vi "Set Cell Data.vi"(4 "Ref. Value":string, 6 "Ref. Header":string, 8 "error in (no error)":errorcluster, 9 "Cell Data":string, 10 "Cell Header":string, 11 "SLL Table in":refnum<class "SLL Table.lvclass">) -> (0 "error out":errorcluster, 3 "SLL Table out":refnum<class "SLL Table.lvclass">)   [LabVIEW 2016, in "SLL Table.lvclass"]
doc: "Set a specific cell value with respect to reference header and value."
uses:
  SLL Table.lvclass
  SLL Table.lvclass/SLL Table.ctl
panel:
  out "Header Present?":bool
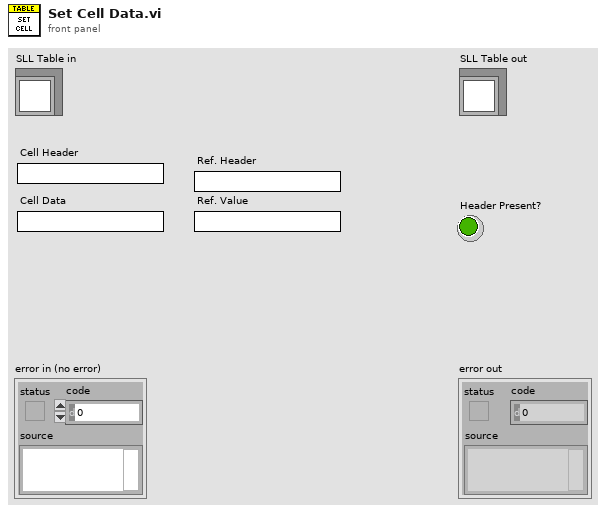
[diagram p1: front panel]
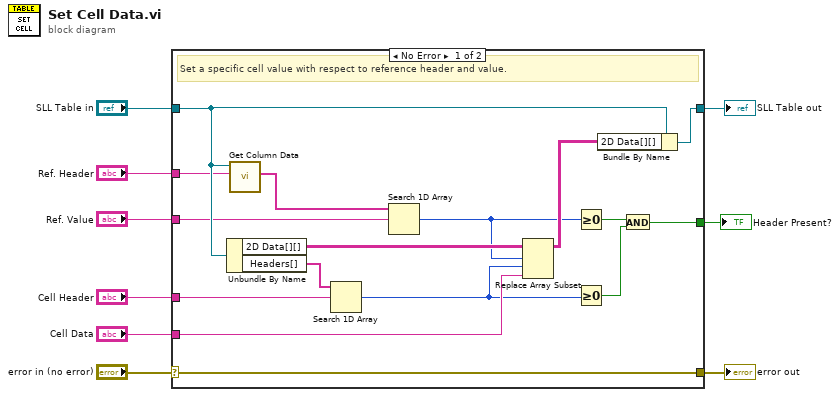
[diagram p0: block diagram]
diagram:
  n1 = case shown="No Error" "error in (no error)" {
    selector: "error in (no error)" -> [w25 w27]
    tunnel: [w25 w27] -> w8
    tunnel: [w18 w26] -> w6
    tunnel: "SLL Table in" -> [w19 w26]
    tunnel: "Cell Header" -> [w22 _]
    tunnel: "Cell Data" -> [w20 _]
    tunnel: "Ref. Header" -> [w16 _]
    tunnel: "Ref. Value" -> [w15 _]
    tunnel: [w10 _] -> w1
    frame No Error {
      # "Set a specific cell value with respect to reference header and value."
      n2 = Unbundle By Name(w19) -> ("2D Data[][]"=w21:string[][], "Headers[]"=w23:string[])
      n3 = call "Get Column Data.vi"("Header"=w16, "SLL Table in"=w19) -> ("Data[]"=w24:string[])  [unwired: 6 in, 3 out]
      n4 = Search 1D Array(1D array=w23, element=w22) -> (index of element=w13:i32)  [unwired: 1 in]
      n5 = Search 1D Array(1D array=w24, element=w15) -> (index of element=w14:i32)  [unwired: 1 in]
      n6 = Replace Array Subset(array=w21, new element=w20, index (row)=w14, index (col)=w13) -> (w17:string[][])
      n7 = Greater Or Equal To 0?(x=w14) -> (x >= 0?=w12:bool)
      n8 = Greater Or Equal To 0?(x=w13) -> (x >= 0?=w11:bool)
      n9 = Bundle By Name(cluster=w19, "2D Data[][]"=w17) -> (w18:refnum<class "SLL Table.lvclass">)
      n10 = And(x=w12, y=w11) -> (x .and. y?=w10:bool)
    }
    frame Error {
    }
  }
  "error out" <- w8
  "SLL Table out" <- w6
  "Header Present?" <- w1
